vi "Stringhandling(SubVI)0.0.2.vi"(0 "Slide (Eingang)":refnum<vi>, 1 "Numerisch (Eingang)":i32, 3 "VISA-Referenz (Eingang)":refnum<visa-resource-name>, 4 "MessFrequenz [Hz]":dbl, 5 "Bytes at Port":u32, 7 "Fehler (Eingang, kein Fehler)":errorcluster, 8 "Cyclecounter (Eingang)":i32, 9 "Rolle[Hz]":dbl, 10 "Temp[°C] (Eingang)":dbl, 11 "AFR (Eingang)":dbl, 12 "String (Eingang)":string, 13 "Zündung [Hz] (Eingang)":dbl, 15 "AFR+EGT":bool) -> (14 "Lesepuffer":string="\n", 16 "Numerisch (Ausgang)":i32, 17 "String (Ausgang)":string, 18 "Temp[°C] (Ausgang)":dbl, 19 "AFR (Ausgang)":dbl, 20 "VISA-Referenz (Ausgang)":refnum<visa-resource-name>, 21 "Zündung [Hz] (Ausgang)":dbl, 23 "Rolle [Hz]":dbl, 24 "Messfrequenz [Hz]":dbl, 25 "Cyclecounter (Ausgang)":i32, 27 "Fehler (Ausgang)":errorcluster)   [LabVIEW 2014]
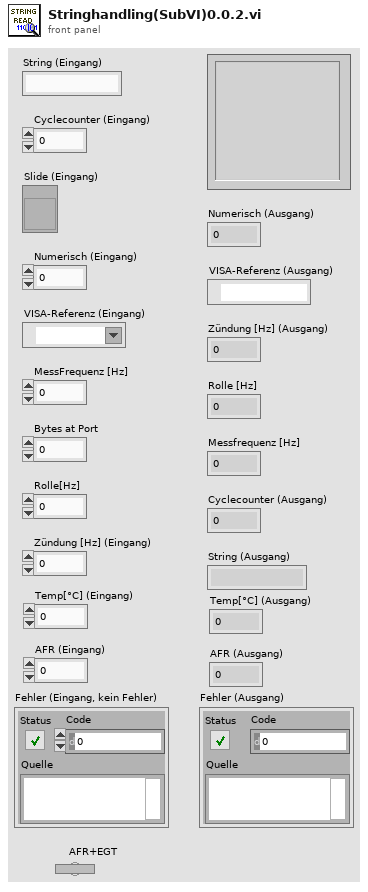
[diagram p1: front panel]
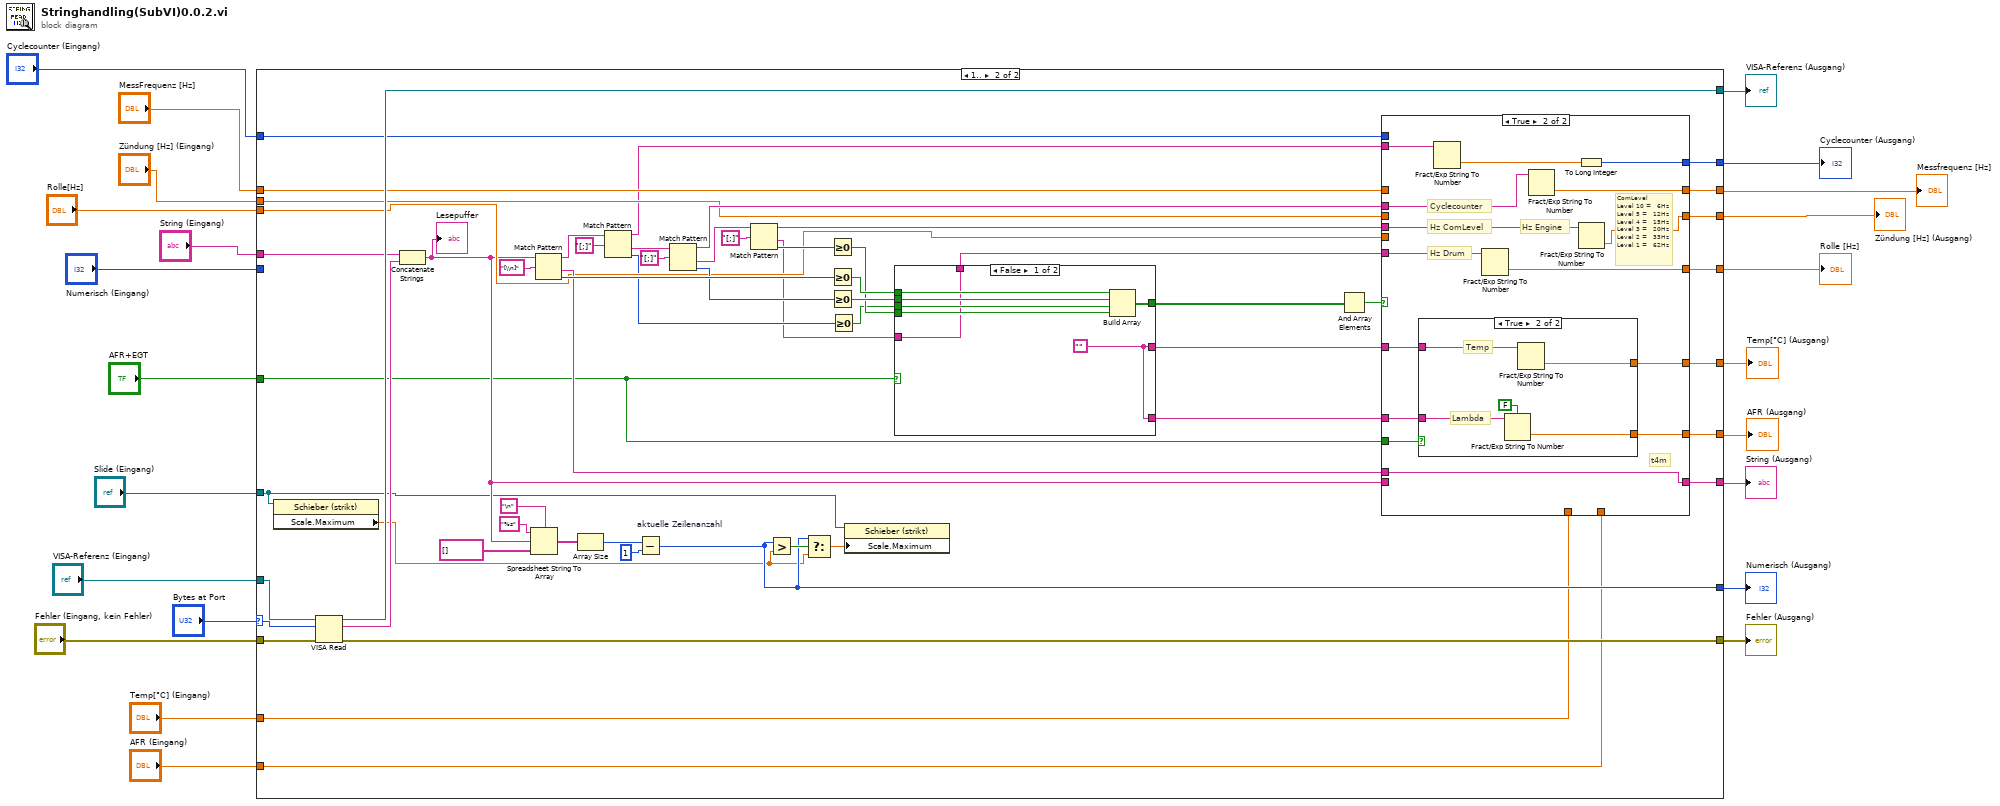
[diagram p0: block diagram]
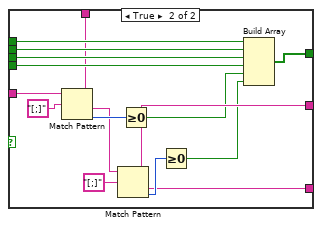
[diagram p3: hidden frame]
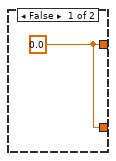
[diagram p5: hidden frame]
diagram:
  n1 = case shown="1.." "Bytes at Port" {
    selector: "Bytes at Port" -> [_ w86]
    tunnel: [w27 w81] -> w15
    tunnel: [w26 w82] -> w20
    tunnel: [w31 w83] -> w13
    tunnel: [w32 w80] -> w12
    tunnel: "String (Eingang)" -> [w33 w78]
    tunnel: [w33 w76] -> w7
    tunnel: "Zündung [Hz] (Eingang)" -> [w32 w68]
    tunnel: "Rolle[Hz]" -> [w31 w67]
    tunnel: [w28 w66] -> w16
    tunnel: "MessFrequenz [Hz]" -> [w28 w65]
    tunnel: "Numerisch (Eingang)" -> [w30 _]
    tunnel: [w30 w48] -> w14
    tunnel: [w29 w54] -> w17
    tunnel: "Cyclecounter (Eingang)" -> [w29 w53]
    tunnel: "VISA-Referenz (Eingang)" -> [w26 w45]
    tunnel: "Fehler (Eingang, kein Fehler)" -> [w27 w44]
    tunnel: "Slide (Eingang)" -> [_ w35]
    tunnel: [w25 w39] -> w5
    tunnel: [w24 w38] -> w4
    tunnel: "Temp[°C] (Eingang)" -> [w25 w37]
    tunnel: "AFR (Eingang)" -> [w24 w36]
    tunnel: "AFR+EGT" -> [_ w34]
    frame 0, Default {
      # "No data in from serial port - Nothing to do."
    }
    frame 1.. {
      n2 = property on="Eigenschaftsknoten" class="Schieber (strikt)"(reference=w35) -> ("Scale.Maximum"=w47:dbl)  [unwired: 1 in, 2 out]
      n3 = VISA Read(VISA resource name=w45, byte count=w86, error in (no error)=w44) -> (VISA resource name out=w82:refnum<visa-resource-name>, read buffer=w79:string, error out=w81:errorcluster)  [unwired: 1 out]
      n4 = Concatenate Strings(w78, w79) -> (w50:string)
      "Lesepuffer" <- w50
      n5 = Spreadsheet String To Array(delimiter (Tab)="\n" ("regular expression"), format string="%s" ("regular expression"), spreadsheet string=w50, array type (2D Dbl)=string[] [] ("Array 2")) -> (array=w59:string[])
      n6 = Match Pattern(string=w50, regular expression="[\\n]") -> (before substring=w57:string, after substring=w77:string, offset past match=w90:i32)  [unwired: 1 in, 1 out]
      n7 = Array Size(array=w59) -> (size(s)=w63:i32)
      n8 = Match Pattern(string=w57, regular expression="[;]") -> (before substring=w55:string, after substring=w56:string, offset past match=w52:i32)  [unwired: 1 in, 1 out]
      n9 = Subtract "aktuelle Zeilenanzahl"(x=w63, y=1) -> (x-y=w48:i32)
      n10 = Match Pattern(string=w56, regular expression="[;]") -> (before substring=w85:string, after substring=w88:string, offset past match=w74:i32)  [unwired: 1 in, 1 out]
      n11 = Match Pattern(string=w88, regular expression="[;]") -> (before substring=w84:string, after substring=w42:string, offset past match=w72:i32)  [unwired: 1 in, 1 out]
      n12 = Greater?(x=w48, y=w47) -> (0:w49:bool)
      n13 = Select(t=w48, s=w49, f=w47) -> (s? t:f=w46:dbl)
      n14 = Greater Or Equal To 0?(x=w72) -> (x >= 0?=w71:bool)
      n15 = Greater Or Equal To 0?(x=w90) -> (x >= 0?=w75:bool)
      n16 = Greater Or Equal To 0?(x=w74) -> (x >= 0?=w73:bool)
      n17 = Greater Or Equal To 0?(x=w52) -> (x >= 0?=w51:bool)
      n18 = property on="Eigenschaftsknoten" class="Schieber (strikt)"(reference=w35, "Scale.Maximum"=w46) -> ()  [unwired: 1 in, 2 out]
      n19 = case shown="False" w34 {
        tunnel: w75 -> [w97 w114]
        tunnel: w73 -> [w96 w113]
        tunnel: w71 -> [w94 w112]
        tunnel: [w98 w111] -> w70
        tunnel: w51 -> [w95 w110]
        tunnel: [w93 w107] -> w43
        tunnel: w42 -> [w93 w106]
        tunnel: [w92 w102] -> w41
        tunnel: [w92 w101] -> w40
        frame False {
          w92 = ""
          n20 = Build Array(w97, w96, w95, w94) -> (w98:bool[])
        }
        frame True {
          n21 = Match Pattern(string=w106, regular expression="[;]") -> (before substring=w107:string, after substring=w103:string, offset past match=w108:i32)  [unwired: 1 in, 1 out]
          n22 = Match Pattern(string=w103, regular expression="[;]") -> (before substring=w101:string, after substring=w102:string, offset past match=w104:i32)  [unwired: 1 in, 1 out]
          n23 = Greater Or Equal To 0?(x=w108) -> (x >= 0?=w100:bool)
          n24 = Greater Or Equal To 0?(x=w104) -> (x >= 0?=w99:bool)
          n25 = Build Array(w114, w113, w110, w112, w100, w99) -> (w111:bool[])
        }
      }
      n26 = And Array Elements(Boolean array=w70) -> (logical AND=w69:bool)
      n27 = case shown="True" w69 {
        tunnel: w85 -> [_ w131]
        tunnel: w84 -> [_ w136]
        tunnel: w43 -> [_ w135]
        tunnel: [w119 w134] -> w83
        tunnel: [w120 w133] -> w80
        tunnel: w77 -> [_ w132]
        tunnel: [w121 w132] -> w76
        tunnel: w50 -> [w121 _]
        tunnel: w68 -> [w120 _]
        tunnel: w67 -> [w119 _]
        tunnel: [w118 w130] -> w66
        tunnel: w65 -> [w118 _]
        tunnel: w55 -> [_ w129]
        tunnel: [w117 w127] -> w54
        tunnel: w53 -> [w117 _]
        tunnel: w41 -> [_ w126]
        tunnel: w40 -> [_ w125]
        tunnel: [w116 w124] -> w39
        tunnel: [w115 w123] -> w38
        tunnel: w37 -> [w116 _]
        tunnel: w36 -> [w115 _]
        tunnel: w34 -> [_ w122]
        frame False {
        }
        frame True {
          # "Cyclecounter"
          # "Hz ComLevel"
          # "ComLevel\nLevel 10 =   6Hz \nLevel 5 =   12Hz \nLevel 4 =   15Hz\nLevel 3 =   20Hz\nLevel 2 =   33Hz\nLevel 1 =   62Hz"
          # "Hz Drum"
          # "Hz Engine"
          # "t4m"
          n28 = case shown="True" w122 {
            tunnel: w126 -> [_ w141]
            tunnel: w125 -> [_ w140]
            tunnel: [w137 w139] -> w124
            tunnel: [w137 w138] -> w123
            frame False {
              w137 = 0.0
            }
            frame True {
              # "Temp"
              # "Lambda"
              n29 = Fract/Exp String To Number(use system decimal point (T)=FALSE, string=w141) -> (number=w138:dbl)  [unwired: 2 in, 1 out]
              n30 = Fract/Exp String To Number(string=w140) -> (number=w139:dbl)  [unwired: 3 in, 1 out]
            }
          }
          n31 = Fract/Exp String To Number(string=w129) -> (number=w128:dbl)  [unwired: 3 in, 1 out]
          n32 = Fract/Exp String To Number(string=w135) -> (number=w134:dbl)  [unwired: 3 in, 1 out]
          n33 = Fract/Exp String To Number(string=w131) -> (number=w130:dbl)  [unwired: 3 in, 1 out]
          n34 = To Long Integer(number=w128) -> (32bit integer=w127:i32)
          n35 = Fract/Exp String To Number(string=w136) -> (number=w133:dbl)  [unwired: 3 in, 1 out]
        }
      }
    }
  }
  "VISA-Referenz (Ausgang)" <- w20
  "Cyclecounter (Ausgang)" <- w17
  "Messfrequenz [Hz]" <- w16
  "Fehler (Ausgang)" <- w15
  "Numerisch (Ausgang)" <- w14
  "Rolle [Hz]" <- w13
  "Zündung [Hz] (Ausgang)" <- w12
  "String (Ausgang)" <- w7
  "AFR (Ausgang)" <- w4
  "Temp[°C] (Ausgang)" <- w5
